vi "select NR Device for 8000A.vi"(8 "error in (no error)":errorcluster, 11 "Anritsu Call Box in":refnum<class "Anritsu Call Box.lvclass">) -> (0 "error out":errorcluster, 3 "Anritsu Call Box out":refnum<class "Anritsu Call Box.lvclass">)   [LabVIEW 2023, in "ANRITSU Call Box.lvlib" / "Anritsu Call Box.lvclass"]
uses:
  Anritsu Call Box.lvclass
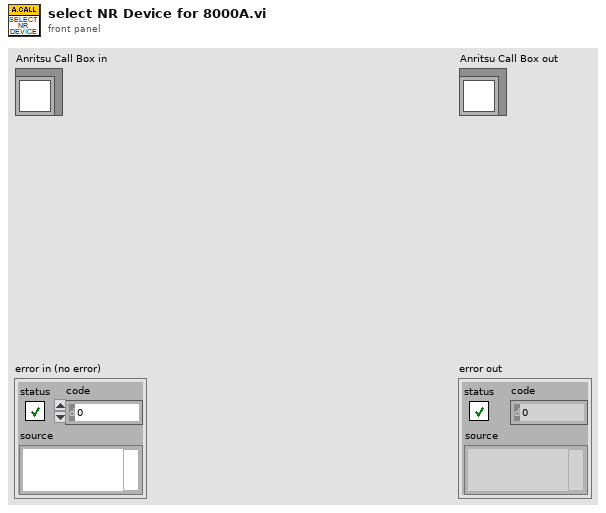
[diagram p1: front panel]
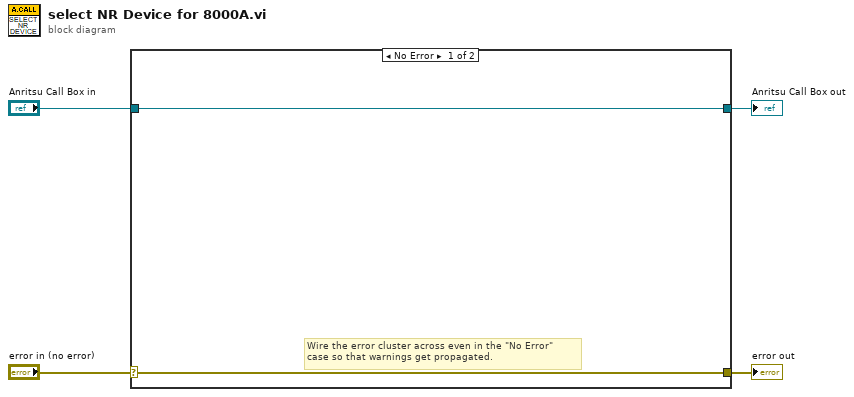
[diagram p0: block diagram]
diagram:
  n1 = case shown="No Error" "error in (no error)" {
    selector: "error in (no error)" -> [w5 w8]
    tunnel: [w5 w8] -> w3
    tunnel: [w6 w7] -> w1
    tunnel: "Anritsu Call Box in" -> [w6 w7]
    frame No Error {
      # "Wire the error cluster across even in the \"No Error\"\ncase so that warnings get propagated."
    }
    frame Error {
    }
  }
  "error out" <- w3
  "Anritsu Call Box out" <- w1
